vi "Test Process Error Handler Configured.vi"(8 "error in (no error)":errorcluster, 11 "Process Test In":refnum<class "Process Test.lvclass">) -> (0 "error out":errorcluster, 3 "Process Test Out":refnum<class "Process Test.lvclass">)   [LabVIEW 2020, in "Process Test.lvclass"]
uses:
  Process Test.lvclass
  C:/Program Files (x86)/National Instruments/LabVIEW 2020/vi.lib/Astemes/LUnit/Test Case.lvclass
  Mock Error Handler/Mock Error Handler.lvclass
  C:/Git/astemes-triarc-framework/source/Framework/Error Handler Interface/Error Handler Interface.lvclass
  Framework/Process/Process.lvclass/Process.ctl
  <vilib>/Astemes/LUnit/Test Case.lvclass/Test Case.ctl
  Framework/Process/Protected/Messaging/Send Message.vi
  Framework/Process/Public/Lifecycle/Get Lifecycle State.vi
  <vilib>/Astemes/LUnit/Palette/Fail.vi
  <vilib>/Astemes/LUnit/Palette/Pass.vi
  <vilib>/Astemes/LUnit/Set Assertion Type.vi
  Framework/Process/Private/SubVIs/Handle Debug Data.vi
  <vilib>/Utility/error.llb/Clear Errors.vi
  <vilib>/Astemes/LUnit/Add test result.vi
  Framework/Logging/Log Debug.vi
  <vilib>/AdvancedString/1D String Array to Delimited String.vi
  <vilib>/Utility/High Resolution Relative Seconds.vi
  <vilib>/Astemes/LUnit/LUnit Record Assertion Result.vi
  <vilib>/Astemes/LUnit/LUnit Aggregate Assertion Results.vi
  <vilib>/Astemes/LUnit/Method Result/LUnit Merge Status.vi
  <vilib>/Astemes/LUnit/LUnit Concatenate result strings.vi
  <vilib>/Utility/error.llb/Error Cluster From Error Code.vi
  Framework/Process/Public/Read Name.vi
  Process Test.lvclass/Process Test.ctl
  Framework/Process/Process.lvclass
  <vilib>/Astemes/LUnit/Test Case.lvclass
  C:/Git/astemes-triarc-framework/source/Framework/Base/Base.lvclass
  C:/Git/astemes-triarc-framework/source/Framework Test Suite/Mock Error Handler/Mock Error Handler.lvclass
  C:/Git/astemes-triarc-framework/source/Framework Test Suite/Base Class Test/Base Test.lvclass
  C:/Git/astemes-triarc-framework/source/Framework Test Suite/Process Test/Process Test.lvclass
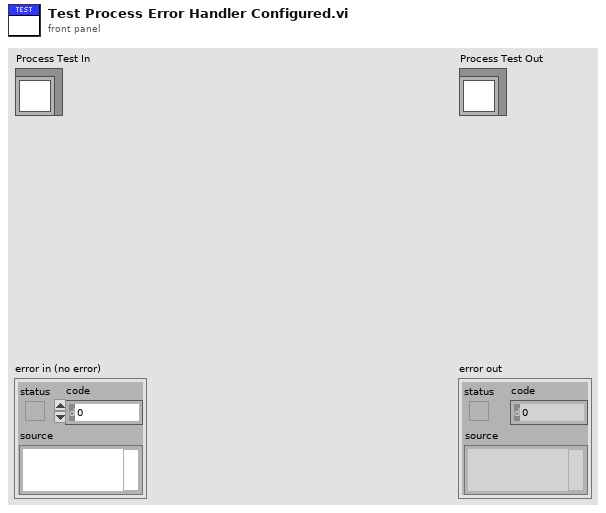
[diagram p1: front panel]
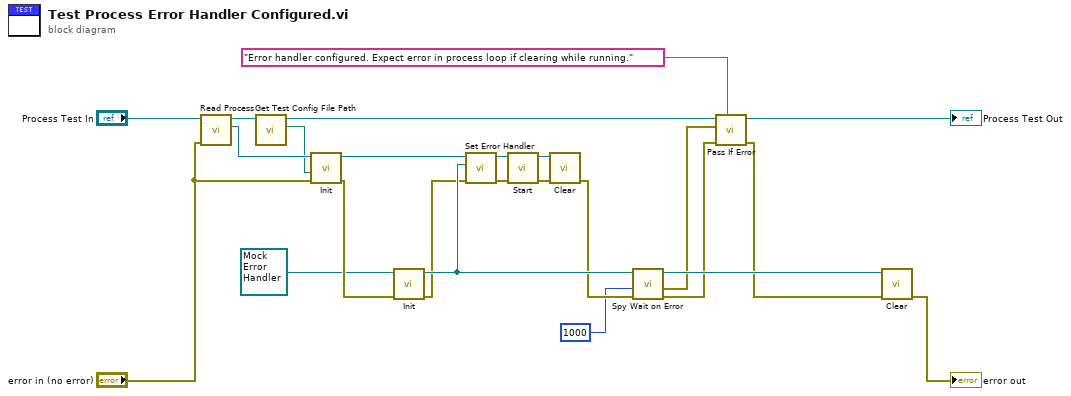
[diagram p0: block diagram]
diagram:
  n1 = call "Read Process.vi"("error in (no error)"="error in (no error)", "Process Test in"="Process Test In") -> ("Process.lvclass"=w12:refnum<class "Process.lvclass">, "Process Test out"=w11:refnum<class "Process Test.lvclass">)  [unwired: 7 in, 1 out]
  n2 = call "Get Test Config File Path.vi"("Process Test In"=w11) -> ("Test config path"=w1:path, "Process Test Out"=w2:refnum<class "Process Test.lvclass">)  [unwired: 8 in, 1 out]
  n3 = call-dynamic "Init.vi"("error in (no error)"="error in (no error)", "Config File Path"=w1, "Process In"=w12) -> ("error out"=w23:errorcluster, "Process Out"=w6:refnum<class "Process.lvclass">)  [unwired: 7 in]
  n4 = call-dynamic "Init.vi"("error in (no error)"=w23, "Mock Error Handler In"=refnum<class "Mock Error Handler.lvclass"> refnum ("Mock Error Handler.lvclass")) -> ("error out"=w7:errorcluster, "Mock Error Handler Out"=w20:refnum<class "Mock Error Handler.lvclass">)  [unwired: 8 in]
  n5 = call "Set Error Handler.vi"("error in (no error)"=w7, "Error Handler"=w20, "Process In"=w6) -> ("error out"=w21:errorcluster, "Process Out"=w4:refnum<class "Process.lvclass">)  [unwired: 7 in]
  n6 = call "Start.vi"("error in (no error)"=w21, "Process In"=w4) -> ("error out"=w5:errorcluster, "Process Out"=w3:refnum<class "Process.lvclass">)  [unwired: 7 in, 1 out]
  n7 = call-dynamic "Clear.vi"("error in (no error)"=w5, "Process In"=w3) -> ("error out"=w17:errorcluster)  [unwired: 9 in]
  n8 = call "Spy Wait on Error.vi"("error in (no error)"=w17, "timeout in ms (-1)"=1000, "Mock Error Handler In"=w20) -> ("error out"=w16:errorcluster, "Errors"=w15:errorcluster, "Mock Error Handler Out"=w19:refnum<class "Mock Error Handler.lvclass">)  [unwired: 4 in, 2 out]
  n9 = call <vilib>:"Pass If Error.vi"("Description"="Error handler configured. Expect error in process loop if clearing while running.", "error in (no error)"=w16, "Assert error"=w15, "LUnit Test Case In"=w2) -> ("error out"=w14:errorcluster, "LUnit Test Case Out"=→"Process Test Out":refnum<class "Process Test.lvclass">)  [unwired: 6 in]
  n10 = call-dynamic "Clear.vi"("error in (no error)"=w14, "Mock Process In"=w19) -> ("error out"=→"error out":errorcluster)  [unwired: 9 in]
